vi "VIH Dialog - Project File List.vi"(4 "Ena Custom VI (F)":bool, 6 "File set (All)":enum32{"ALL", "conpane", "invalid"}(ring), 7 "Called from Master (F)":bool, 10 "Disable not buildable":bool, 11 "Project Tree":T2) -> (0 "OK out":bool, 2 "File Paths":path[](array[path]), 3 "File Path":path)   [LabVIEW 2014]
doc: "::: VI Helpeks :::\nCopyright (c) 2000-2026 Konstantin Shifershteyn. All rights reserved."
uses:
  VIH Project Tree Typedef - Tree Refnum.ctl
  _VIH HelpGen - Palette.llb/VIH HelpGen Typedef - Palette - Item Type Enum.ctl
  VIH Project Tree Typedef - Tree Item Type.ctl
  <vilib>/Utility/miscctls.llb/LVRowAndColumnUnsignedTypeDef.ctl
panel:
  in  "QualifiedNames":bool caption="Show qualified VI names"
  in  "KindOfFile":T1(ring) caption="Category Selector"
  in  "Files w NotFound Attrib":path[](array[path])
  in  "DirectSortColumn":i32
  in  "Files tmp":path[](array[path])
  in  "FileList":i32[](listbox) caption="File List"
  out "Sel Path":path caption="File Path"
  in  "%Arbitrary":bool caption="Custom VI"
  in  "%OK":bool caption="OK"
  in  "%Cancel":bool caption="Cancel"
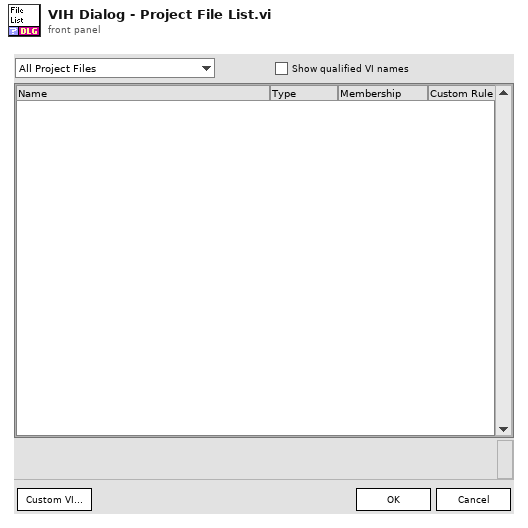
[diagram p1: front panel]
types:
  T1 = enum16{"All Project Files", "Palette menus", "Instruments (VI,VIT)", "VIs with Connector Pane", "Express VIs", "Polymorphic VIs", "Controls (CTL,CTT)", "HTML Files", "Other Files", "Invalid Files"}
  T2 = typedef "VIH Project Tree Typedef - Tree Refnum.ctl" = refnum<vi>
  T3 = typedef "VIH HelpGen Typedef - Palette - Item Type Enum.ctl" = enum32{"<Invalid>", "<unknown>", "VI", "Menu", "LV Func", "Express VI", "Poly VI", "CTL", "HTML"}
  T4 = cluster{"Types":T3[], "Paths":path[], "Dynamic":enum16{"Dyn", "Stat", "Both"}[], "Can be built":bool[], "Has rule":bool[], "Names":string[]}
  T5 = enum8{"Enabled", "Disabled", "Disabled and Grayed Out"}
  T6 = typedef "VIH Project Tree Typedef - Tree Item Type.ctl" = enum32{"<Invalid>", "Project", "Proj Files", "Proj Rules", "File Group", "Rule Group", "Any File", "LV Func", ".mnu", ".mnu (dyn)", ".vi", ".vi (dyn)", ".vit", ".vit (dyn)", ".ctl", ".ctl (dyn)", ".ctt", ".ctt (dyn)", "polyVI", "polyVI (dyn)", "expVI", "expVI (dyn)", "HTML", "PolyVI Inst"}
  T7 = typedef "LVRowAndColumnUnsignedTypeDef.ctl" = cluster{"Row":u32, "Column":u32}
  T8 = typedef "LVPoint32TypeDef.ctl" = cluster{"Horizontal":i32, "Vertical":i32}
  T9 = typedef "LVRowAndColumnTypeDef.ctl" = cluster{"Row":i32, "Column":i32}
  T10 = typedef "lveventtype.ctl" = enum32{"Null", "Timeout", "Annotation Menu Selection", "Annotation Menu Selection?", "App Instance Close", "App Instance Close?", "Autoscale Range Change", "Bookmark Info Change", "Cell Edit", "Cell Edit?", "Cursor Grab", "Cursor Grab?", "Cursor Menu Selection", "Cursor Menu Selection?", "Cursor Move", "Cursor Release", "Data Change", "Direction Change", "Display State Change", "Drag Ended", "Drag Enter", "Drag Leave", "Drag Over", "Drag Source Update", "Drag Starting", "Drag Starting?", "Drop", "Exec State Change", "Key Down", "Key Down?", "Key Repeat", "Key Repeat?", "Key Up", "Listbox Double Click", "Menu Activation?", "Menu Selection (App)", "Menu Selection? (App)", "Menu Selection (User)", "Mouse Down", "Mouse Down?", "Mouse Enter", "Mouse Leave", "Mouse Move", "Mouse Up", "Mouse Wheel", "NI Security User Change (App)", "Pane Size", "Panel Close", "Panel Close?", "Panel Resize", "Plot Attribute Change", "Scale Range Change", "Shortcut Menu Activation?", "Shortcut Menu Selection (App)", "Shortcut Menu Selection? (App)", "Shortcut Menu Selection (User)", "Tree Double Click", "Tree Drag", "Tree Drag?", "Tree Drop", "Tree Drop?", "Tree Item Close", "Tree Item Close?", "Tree Item Open", "Tree Item Open?", "User Event", "Value Change"}
  T11 = cluster{"Types":T3[], "Paths":path[], "Dynamic":enum16{"Dyn", "Stat", "Both"}[], "Can be built":bool[], "DynFileNotFound":bool[]}
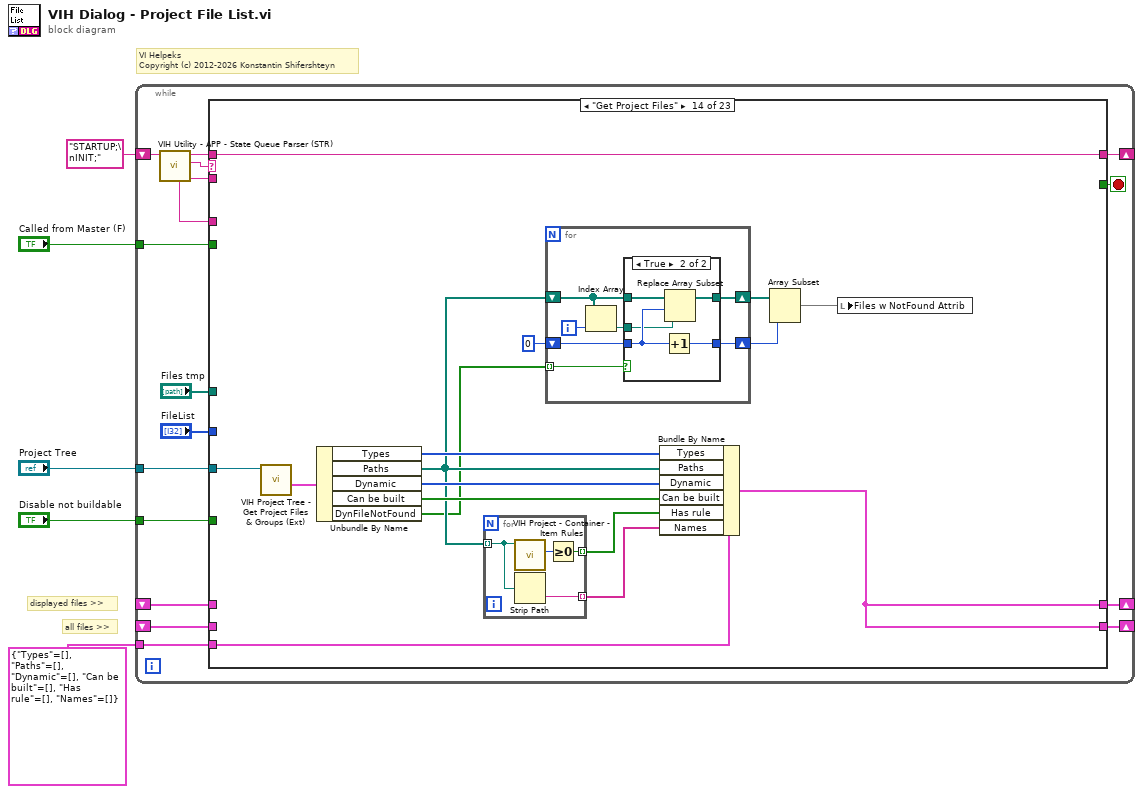
[diagram p0: block diagram]
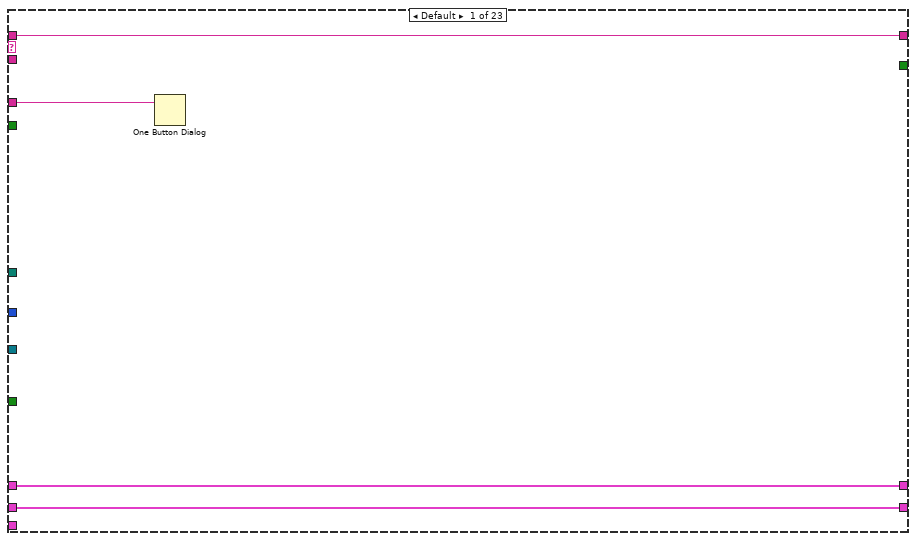
[diagram p2: hidden frame]
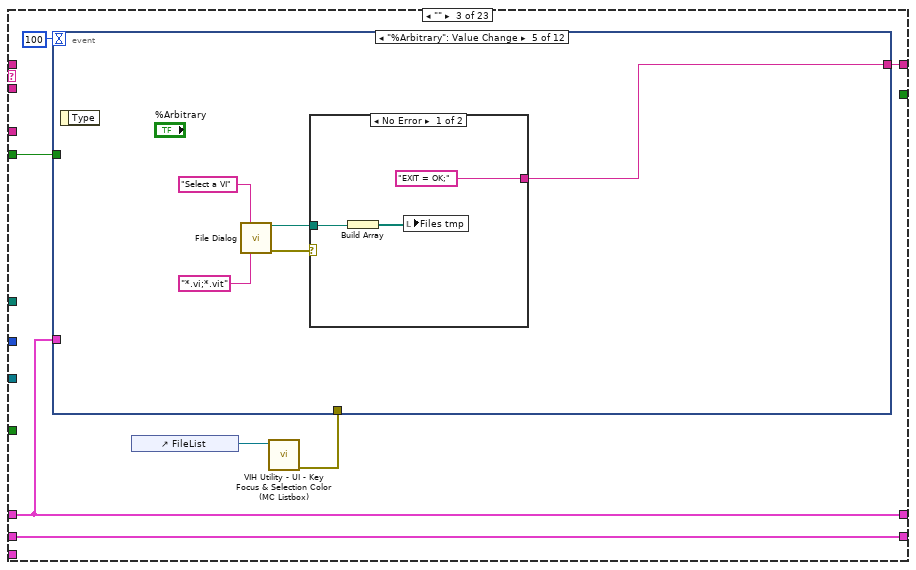
[diagram p4: hidden frame]
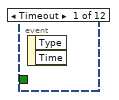
[diagram p5: hidden frame]
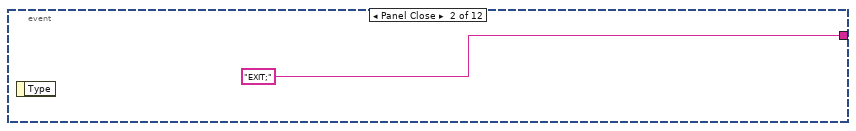
[diagram p6: hidden frame]
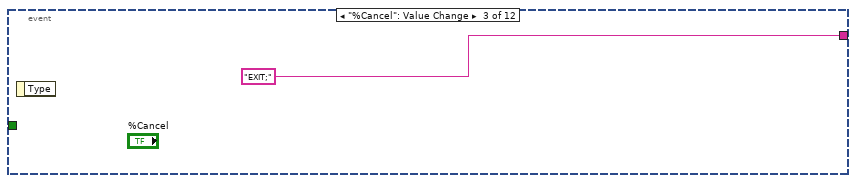
[diagram p7: hidden frame]
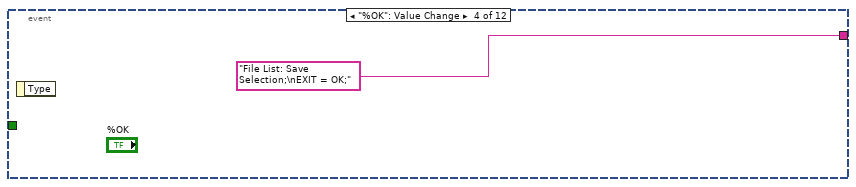
[diagram p8: hidden frame]
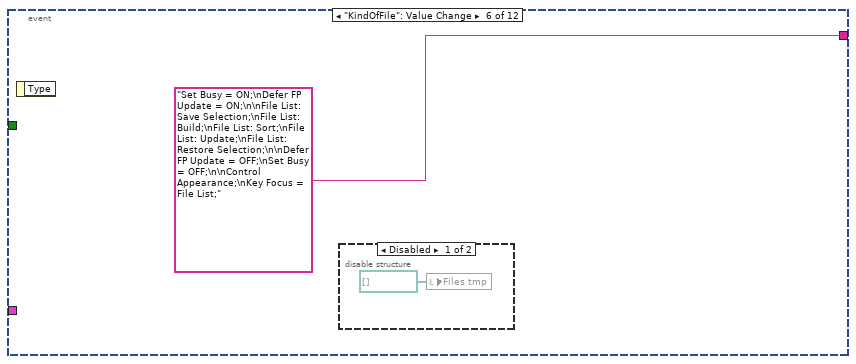
[diagram p10: hidden frame]
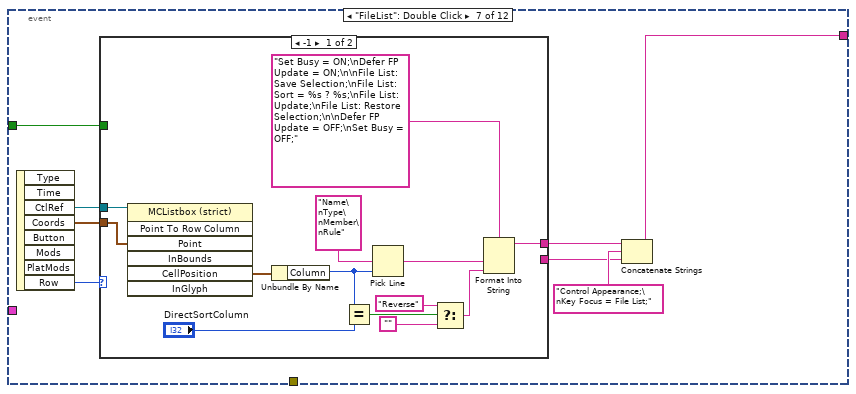
[diagram p12: hidden frame]
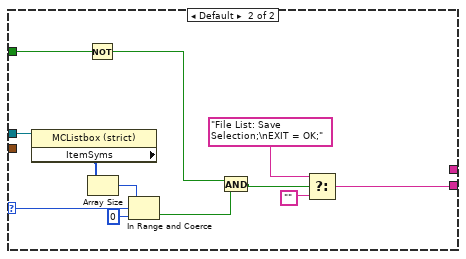
[diagram p13: hidden frame]
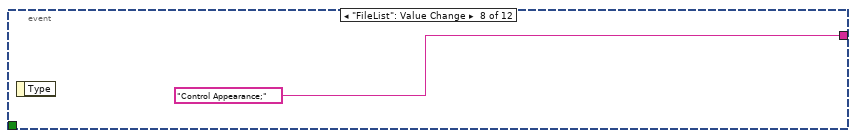
[diagram p14: hidden frame]
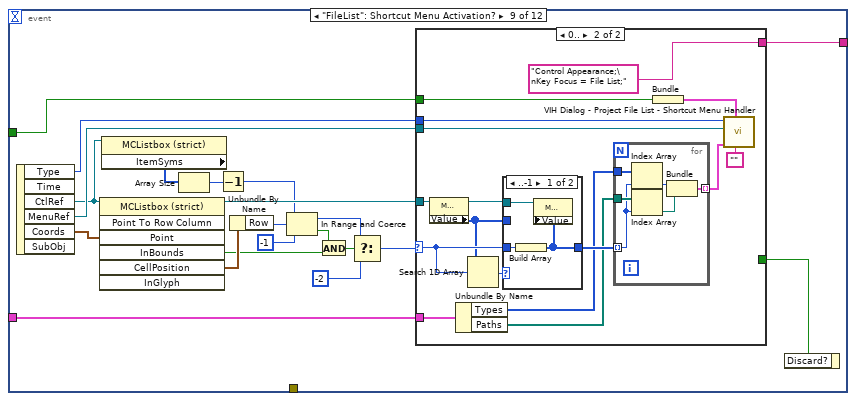
[diagram p15: hidden frame]
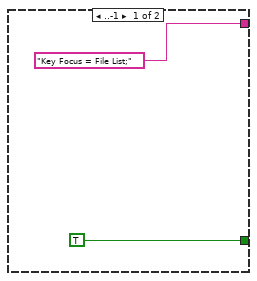
[diagram p16: hidden frame]
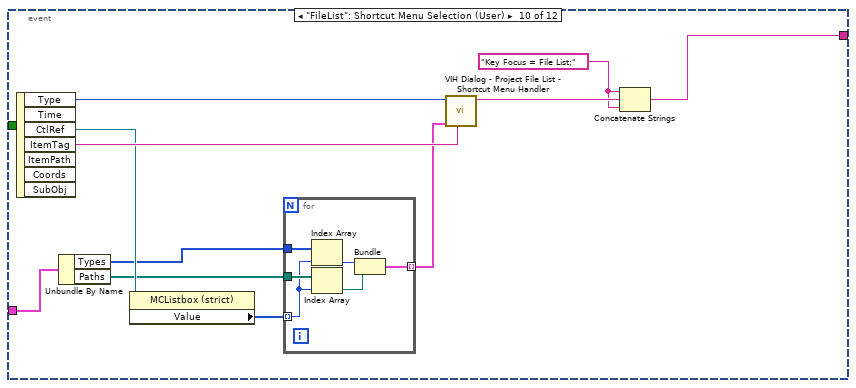
[diagram p18: hidden frame]
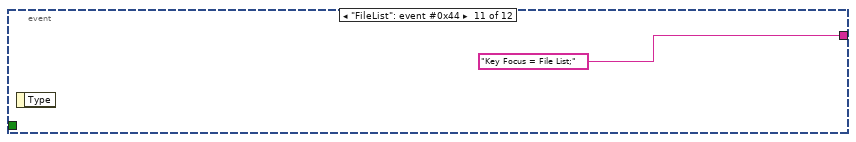
[diagram p19: hidden frame]
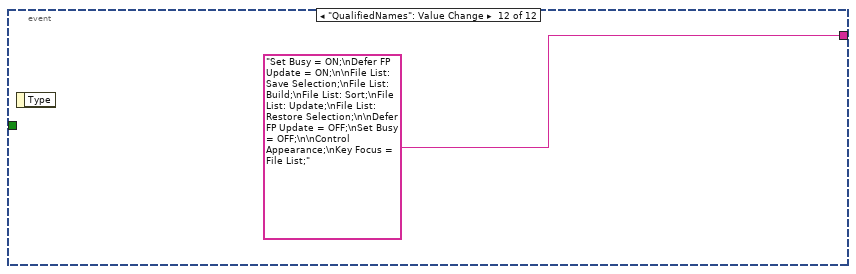
[diagram p20: hidden frame]
diagram:
  # "VI Helpeks\nCopyright (c) 2012-2026 Konstantin Shifershteyn"
  # "displayed files >>"
  # "all files >>"
  n1 = while {
    shift-right: [w20] -> _
    shift-left: "STARTUP;\nINIT;" -> [w22]
    tunnel: "Project Tree" -> [w15]
    shift-right: [w14] -> _
    shift-left: _ -> [w13]
    shift-right: [w12] -> _
    shift-left: _ -> [w11]
    tunnel: T4 {"Types"=[], "Paths"=[], "Dynamic"=[], "Can be built"=[], "Has rule"=[], "Names"=[]} ("Project Files") -> [w8]
    tunnel: "Called from Master (F)" -> [w7]
    tunnel: "Disable not buildable" -> [w6]
    stop <- w17 stop-if-true
    n2 = call "VIH Utility - APP - State Queue Parser (STR).vi"("input queue"=w22) -> ("state parameters"=w16:string, "state"=w21:string, "remained queue"=w19:string, "complete state specifier"=w18:string)  [unwired: 5 in]
    n3 = case shown="\"Get Project Files\"" w21 {
      tunnel: [w26 w29 w35 w153 w190 "File List: Clear;\nHALT;" w223 w237 w241 w247 w252 w264 w273 w289 w334 w453 w647 w717 w736 w756 w760 w767 w797] -> w20
      tunnel: w19 -> [w26 w29 _ w156 w191 _ w223 w237 w241 w247 w252 w264 w273 w289 w334 w453 w647 w717 w736 w756 w760 w775 w803]
      tunnel: w18 -> [w25 _ _ _ _ _ _ _ _ _ _ _ _ _ _ _ _ _ _ _ _ _ _]
      tunnel: [_ _ _ _ _ _ TRUE _ _ _ _ _ _ _ _ _ _ _ _ _ _ _ _] -> w17
      tunnel: w16 -> [_ _ _ _ _ w203 _ _ w238 w242 w249 _ _ _ _ w439 _ _ _ _ _ w771 w790]
      tunnel: w15 -> [_ _ _ _ _ _ _ _ _ _ _ _ _ w288 _ _ _ _ _ _ _ w772 w800]
      tunnel: [w24 w28 w34 w158 w188 w201 w221 w235 w239 w245 w250 w263 w271 w284 w333 w454 w648 w718 w737 w757 w758 w773 w801] -> w14
      tunnel: w13 -> [w24 w28 w34 w158 w188 w201 _ w235 w239 w245 w250 w263 w271 _ w333 w454 w648 w718 w737 w757 w758 w773 w801]
      tunnel: [w23 w27 w33 w157 w187 w198 w221 w236 w240 w246 w251 w262 w272 w284 w326 w447 w646 w716 w735 w755 w759 w774 w802] -> w12
      tunnel: w11 -> [w23 w27 w33 w157 w187 w198 _ w236 w240 w246 w251 w262 w272 _ _ w452 w646 w716 w735 w755 w759 w774 w802]
      tunnel: "FileList" -> [_ _ _ _ _ w197 _ _ _ _ _ w261 _ _ _ _ _ w715 _ _ _ _ _]
      tunnel: "Files tmp" -> [_ _ _ _ _ w200 _ _ _ _ _ _ _ _ _ _ _ _ w722 _ _ _ _]
      tunnel: w8 -> [_ _ _ _ _ _ w221 _ _ _ _ _ _ w286 w319 w444 _ _ _ _ _ _ _]
      tunnel: w7 -> [_ _ w32 _ w173 _ _ _ _ _ _ w257 _ _ _ _ _ _ _ _ _ _ _]
      tunnel: w6 -> [_ _ _ _ _ _ _ _ _ _ _ _ _ _ _ _ w632 _ _ _ _ _ _]
      frame Default {
        n4 = One Button Dialog(message=w25) -> ()  [unwired: 1 in, 1 out]
      }
      frame "#" {
      }
      frame "" {
        n5 = control-ref of="FileList"() -> (w31:refnum<vi>)
        n6 = call "VIH Utility - UI - Key Focus & Selection Color (MC Listbox).vi"("MCListbox Refnum"=w31) -> ("error out"=w30:errorcluster)  [unwired: 8 in, 2 out]
        n7 = event shown="[4] \"%Arbitrary\": Value Change" {
          selector: _ -> [_ _ _ _ _ _ _ _ _ _ _ _]
          dyn-events: _ -> [_ _ _ _ _ _ _ _ _ _ _ _]
          timeout: 100 -> [_ _ _ _ _ _ _ _ _ _ _ _]
          tunnel: [_ "EXIT;" "EXIT;" "File List: Save Selection;\nEXIT = OK;" w40 "Set Busy = ON;\nDefer FP Update = ON;\n\nFile List: Save Selection;\nFile List: Build;\nFile List: Sort;\nFile List: Update;\nFile List: Restore Selection;\n\nDefer FP Update = OFF;\nSet Busy = OFF;\n\nControl Appearance;\nKey Focus = File List;" w53 "Control Appearance;" w87 w136 "Key Focus = File List;" ("string") "Set Busy = ON;\nDefer FP Update = ON;\n\nFile List: Save Selection;\nFile List: Build;\nFile List: Sort;\nFile List: Update;\nFile List: Restore Selection;\n\nDefer FP Update = OFF;\nSet Busy = OFF;\n\nControl Appearance;\nKey Focus = File List;"] -> w35
          tunnel: w33 -> [_ _ _ _ _ _ _ _ w96 w138 _ _]
          tunnel: w32 -> [_ _ _ _ _ _ w50 _ w95 _ _ _]
          tunnel: w30 -> [_ _ _ _ _ _ _ _ _ _ _ _]
          event Timeout {
            n8 = event-data() -> ()  [unwired: 1 in, 2 out]
          }
          event Panel Close {
            n9 = event-data() -> ()  [unwired: 1 in, 1 out]
          }
          event "%Cancel": Value Change {
            n10 = event-data() -> ()  [unwired: 1 in, 1 out]
          }
          event "%OK": Value Change {
            n11 = event-data() -> ()  [unwired: 1 in, 1 out]
          }
          event "%Arbitrary": Value Change {
            n12 = event-data() -> ()  [unwired: 1 in, 1 out]
            n13 = call "File Dialog"("prompt"="Select a VI", "pattern (all files)"="*.vi;*.vit") -> ("selected path"=w41:path, "error out"=w42:errorcluster)  [unwired: 10 in, 2 out]
            n14 = case shown="No Error" w42 {
              tunnel: w41 -> [w47 _]
              tunnel: ["EXIT = OK;" _] -> w40
              frame No Error {
                n15 = Build Array(w47) -> (w46:path[])
                n16 = local write "Files tmp"(w46) -> ()
              }
              frame Error {
              }
            }
          }
          event "KindOfFile": Value Change {
            n17 = event-data() -> ()  [unwired: 1 in, 1 out]
            n18 = disable-structure shown="Disabled" {
              frame Disabled {
                n19 = local write "Files tmp"(path[] [] ("Files tmp")) -> ()
              }
              frame Enabled {
              }
            }
          }
          event "FileList": Double Click {
            n20 = event-data() -> ("CtlRef"=w56:refnum<vi>, "Coords"=w55:T8, "Row"=w57:i32)  [unwired: 1 in, 5 out]
            n21 = case shown="-1" w57 {
              selector: w57 -> [_ w81]
              tunnel: w56 -> [w70 w82]
              tunnel: w55 -> [w69 _]
              tunnel: [w64 _] -> w54
              tunnel: [_ w77] -> w51
              tunnel: w50 -> [_ w72]
              frame -1 {
                n22 = invoke class="MCListbox (strict)" method="Point To Row Column"(reference=w70, "Point"=w69) -> ("CellPosition"=w68:T9)  [unwired: 5 in, 6 out]
                n23 = Unbundle By Name(w68) -> ("Column"=w62:i32)
                n24 = Equal?(x=w62, y="DirectSortColumn") -> (x = y?=w61:bool)
                n25 = Pick Line(multi-line string="Name\nType\nMember\nRule", line index=w62) -> (output string=w65:string)  [unwired: 1 in]
                n26 = Select(t="Reverse", s=w61, f="") -> (s? t:f=w59:string)
                n27 = Format Into String(format string="Set Busy = ON;\nDefer FP Update = ON;\n\nFile List: Save Selection;\nFile List: Sort = %s ? %s;\nFile List: Update;\nFile List: Restore Selection;\n\nDefer FP Update = OFF;\nSet Busy = OFF;", w65, w59) -> (resulting string=w64:string)  [unwired: 2 in, 1 out]
              }
              frame Default {
                n28 = property class="MCListbox (strict)"(reference=w82) -> ("ItemSyms"=w80:i32[])  [unwired: 1 in, 2 out]
                n29 = Not(x=w72) -> (.not. x?=w71:bool)
                n30 = Array Size(array=w80) -> (size(s)=w79:i32)
                n31 = In Range and Coerce(upper limit=w79, x=w81, lower limit=0) -> (In Range?=w73:bool)  [unwired: 1 out]
                n32 = And(x=w71, y=w73) -> (x .and. y?=w74:bool)
                n33 = Select(t="File List: Save Selection;\nEXIT = OK;", s=w74, f="") -> (s? t:f=w77:string)
              }
            }
            n34 = Concatenate Strings(w54, "Control Appearance;\nKey Focus = File List;", w51) -> (w53:string)
          }
          event "FileList": Value Change {
            n35 = event-data() -> ()  [unwired: 1 in, 1 out]
          }
          event "FileList": Shortcut Menu Activation? {
            n36 = event-data() -> ("Type"=w98:T10, "CtlRef"=w94:refnum<vi>, "MenuRef"=w97:refnum<k9>, "Coords"=w104:T8)  [unwired: 1 in, 2 out]
            n37 = invoke class="MCListbox (strict)" method="Point To Row Column"(reference=w94, "Point"=w104) -> (reference out=w99:refnum<vi>, "InBounds"=w85:bool, "CellPosition"=w103:T9)  [unwired: 5 in, 4 out]
            n38 = property class="MCListbox (strict)"(reference=w94) -> ("ItemSyms"=w92:i32[])  [unwired: 1 in, 2 out]
            n39 = Array Size(array=w92) -> (size(s)=w91:i32)
            n40 = Decrement(x=w91) -> (x-1=w90:i32)
            n41 = Unbundle By Name(w103) -> ("Row"=w93:i32)
            n42 = In Range and Coerce(upper limit=w90, x=w93, lower limit=-1) -> (coerced(x)=w88:i32, In Range?=w86:bool)
            n43 = And(x=w86, y=w85) -> (x .and. y?=w84:bool)
            n44 = Select(t=w88, s=w84, f=-2) -> (s? t:f=w101:i32)
            n45 = case shown="0.." w101 {
              selector: w101 -> [_ w119]
              tunnel: [TRUE _] -> w100
              tunnel: w99 -> [_ w122]
              tunnel: w98 -> [_ w118]
              tunnel: w97 -> [_ w117]
              tunnel: w96 -> [_ w112]
              tunnel: w95 -> [_ w111]
              tunnel: ["Key Focus = File List;" "Control Appearance;\nKey Focus = File List;"] -> w87
              frame ..-1 {
              }
              frame 0.. {
                n46 = property class="MCListbox (strict)"(reference=w122) -> (reference out=w121:refnum<vi>, "Value"=w115:i32[])  [unwired: 1 in, 1 out]
                n47 = Unbundle By Name(w112) -> ("Types"=w109:T3[], "Paths"=w113:path[])
                n48 = Search 1D Array(1D array=w115, element=w119) -> (index of element=w120:i32)  [unwired: 1 in]
                n49 = case shown="..-1" w120 {
                  tunnel: w121 -> [w131 _]
                  tunnel: w119 -> [w130 _]
                  tunnel: [w129 w132] -> w114
                  tunnel: w115 -> [_ w132]
                  frame ..-1 {
                    n50 = Build Array(w130) -> (w129:i32[])
                    n51 = property class="MCListbox (strict)"(reference=w131, "Value"=w129) -> ()  [unwired: 1 in, 2 out]
                  }
                  frame 0.. {
                  }
                }
                n52 = for {
                  tunnel: w114 -> [w126] mode=indexing
                  tunnel: w113 -> [w128]
                  tunnel: w109 -> [w127]
                  tunnel: [w123] -> w108 mode=indexing
                  n53 = Index Array(array=w127, index=w126) -> (element=w125:T3)
                  n54 = Index Array(array=w128, index=w126) -> (element=w124:path)
                  n55 = Bundle("Item/File Type"=w125, w124) -> (w123:cluster{"Item/File Type":T3, path})  [unwired: 1 in]
                }
                n56 = Bundle("Called from Master (F)"=w111) -> (w110:cluster{"Called from Master (F)":bool})  [unwired: 1 in]
                n57 = call "VIH Dialog - Project File List - Shortcut Menu Handler.vi"("Menu Tag"="", "Options"=w110, "Files"=w108, "MenuRef"=w117, "Event Type"=w118) -> ()  [unwired: 6 in, 1 out]
              }
            }
            n58 = event-data("Discard?"=w100) -> ()  [unwired: 1 in, 1 out]
          }
          event "FileList": Shortcut Menu Selection (User) {
            w133 = "Key Focus = File List;" ("string")
            n59 = event-data() -> ("Type"=w143:T10, "CtlRef"=w140:refnum<vi>, "ItemTag"=w141:string)  [unwired: 1 in, 4 out]
            n60 = Unbundle By Name(w138) -> ("Types"=w135:T3[], "Paths"=w137:path[])
            n61 = property class="MCListbox (strict)"(reference=w140) -> ("Value"=w139:i32[])  [unwired: 1 in, 2 out]
            n62 = for {
              tunnel: w139 -> [w144] mode=indexing
              tunnel: w137 -> [w149]
              tunnel: w135 -> [w148]
              tunnel: [w145] -> w134 mode=indexing
              n63 = Index Array(array=w148, index=w144) -> (element=w147:T3)
              n64 = Index Array(array=w149, index=w144) -> (element=w146:path)
              n65 = Bundle("Item/File Type"=w147, w146) -> (w145:cluster{"Item/File Type":T3, path})  [unwired: 1 in]
            }
            n66 = call "VIH Dialog - Project File List - Shortcut Menu Handler.vi"("Menu Tag"=w141, "Files"=w134, "Event Type"=w143) -> ("States spec"=w142:string)  [unwired: 8 in]
            n67 = Concatenate Strings(w133, w142, w133) -> (w136:string)
          }
          event "FileList": event #0x44 {
            n68 = event-data() -> ()  [unwired: 1 in, 1 out]
          }
          event "QualifiedNames": Value Change {
            n69 = event-data() -> ()  [unwired: 1 in, 1 out]
          }
        }
      }
      frame "STARTUP" {
        n70 = control-ref of="FileList"() -> (w155:refnum<vi>)
        n71 = disable-structure shown="Disabled" {
          disable-tunnel: w155 -> [w161 _]
          disable-tunnel: "Utility - Set Project Tree & List Icons.vi" ("Utility VI Name") -> [w160 _]
          frame Disabled {
            n72 = call "VIH Utility - DEV - Get DevTime Utility VIs Folder.vi"("Utility VI Name"=w160) -> ("error out"=w167:errorcluster, "Utility VIs Path"=w166:path)  [unwired: 8 in, 1 out]
            n73 = Open VI Reference(type specifier VI Refnum (for type only)=refnum<vi> refnum, vi path=w166, error in (no error)=w167) -> (vi reference=w169:refnum<vi>, error out=w170:errorcluster)  [unwired: 3 in]
            n74 = call-by-ref "?"(reference=w169, error in=w170, "MCListbox Refnum"=w161) -> (reference out=w164:refnum<vi>, error out=w165:errorcluster, "error out (MCList)"=w162:errorcluster)  [unwired: 9 in, 1 out]
            n75 = Close Reference(reference=w164, error in (no error)=w165) -> (error out=w159:errorcluster)
            n76 = Select(t=w159, s=w159, f=w162) -> (s? t:f=w163:errorcluster)
            n77 = call <vilib>:"Simple Error Handler.vi"("error in (no error)"=w163) -> ()  [unwired: 4 in, 5 out]
          }
          frame Enabled {
          }
        }
        n78 = Concatenate Strings("File List: Clear;" ("string"), w156) -> (w153:string)
      }
      frame "INIT" {
        w171 = path[] [] ("Files tmp")
        n79 = call "VIH Utility - UI - Boolean to Control Disable Status.vi"("Status in"="Ena Custom VI (F)") -> ("Control Disable if False"=w185:u8)  [unwired: 3 in, 1 out]
        n80 = Not(x=w173) -> (.not. x?=w174:bool)
        n81 = property on="%Arbitrary" class="Bool"("DisabledEnum"=w185, "Visible"="Ena Custom VI (F)") -> ()  [unwired: 2 in, 2 out]
        n82 = property on="%OK" class="Bool"("Visible"=w174) -> ()  [unwired: 2 in, 2 out]
        n83 = Select(t="Close", s=w173, f="Cancel") -> (s? t:f=w180:string)
        n84 = case shown="\"invalid\"" "File set (All)" {
          tunnel: [T1."All Project Files" ("KindOfFile") T1."VIs with Connector Pane" ("KindOfFile") T1."Invalid Files" ("KindOfFile")] -> w184
          tunnel: [_ T5."Disabled and Grayed Out" ("Disabled") _] -> w183
          frame "ALL" {
          }
          frame "conpane" {
          }
          frame "invalid" {
          }
        }
        n85 = Initialize Array(w180, 4 ("dimension size")) -> (w179:string[])
        n86 = Select(t="Project Files", s=w173, f="Select a Project File") -> (s? t:f=w175:string)
        n87 = local write "Files w NotFound Attrib"(w171) -> ()
        n88 = local write "Files tmp"(w171) -> ()
        n89 = property on="%Cancel" class="Bool"("Strings [4]"=w179) -> ()  [unwired: 2 in, 2 out]
        n90 = property class="VI"("Front Panel.Title"=w175) -> ()  [unwired: 2 in, 2 out]
        n91 = property on="KindOfFile" class="Enum (strict)"("DisabledEnum"=w183, "Value"=w184) -> ()  [unwired: 2 in, 2 out]
        n92 = Concatenate Strings("Set Busy = ON;\nDefer FP Update = ON;\n\nGet Project Files;\n\nFile List: Build;\nFile List: Sort;\nFile List: Update;\nFile List: Restore Selection;\n\nDefer FP Update = OFF;\nSet Busy = OFF;\n\nControl Appearance;\nKey Focus = File List;", w191) -> (w190:string)
      }
      frame "EXIT" {
        n93 = case shown="\"Find In Tree\"" w203 {
          tunnel: [_ TRUE TRUE] -> w202
          tunnel: w200 -> [_ w206 w213]
          tunnel: [_ w205 w212] -> w199
          tunnel: w198 -> [_ _ w211]
          tunnel: w197 -> [_ _ w209]
          tunnel: [_ _ w208] -> w196
          frame Default {
          }
          frame "OK" {
            n94 = Index Array(array=w206) -> (element=w205:path)  [unwired: 1 in]
          }
          frame "Find In Tree" {
            n95 = Unbundle By Name(w211) -> ("Paths"=w210:path[])
            n96 = Index Array(array=w213) -> (element=w212:path)  [unwired: 1 in]
            n97 = for {
              tunnel: w210 -> [w217]
              tunnel: w209 -> [w216] mode=indexing
              tunnel: [w215] -> w208 mode=indexing
              n98 = Index Array(array=w217, index=w216) -> (element=w215:path)
            }
          }
        }
        "OK out" <- w202
        "File Path" <- w199
        "File Paths" <- w196
      }
      frame "HALT" {
        n99 = Call Chain() -> (call chain=w220:string[])
        n100 = Array Size(array=w220) -> (size(s)=w219:i32)
        n101 = case shown="2.." w219 {
          tunnel: [_ TRUE] -> w218
          frame ..1 {
          }
          frame 2.. {
            n102 = for {
              N: 100 -> [_]
              stop <- w233 continue-if-true
              n103 = property class="VI"("Front Panel.Open"=FALSE ("Front Panel Window:Open")) -> ("Front Panel.Open"=w233:bool)  [unwired: 2 in, 2 out]
              n104 = Wait (ms)(milliseconds to wait=u32 10) -> ()  [unwired: 1 out]
            }
          }
        }
        n105 = stacked-sequence {
          tunnel: w218 -> [_]
          frame #0 {
            w224 = T5."Enabled" ("Disabled")
            w226 = TRUE ("Visible")
            n106 = Initialize Array("Cancel", 4 ("dimension size")) -> (w228:string[])
            n107 = property on="%OK" class="Bool"("DisabledEnum"=w224, "Visible"=w226) -> ()  [unwired: 2 in, 2 out]
            n108 = property on="%Cancel" class="Bool"("Strings [4]"=w228) -> ()  [unwired: 2 in, 2 out]
            n109 = property on="%Arbitrary" class="Bool"("DisabledEnum"=w224, "Visible"=w226) -> ()  [unwired: 2 in, 2 out]
            n110 = property on="KindOfFile" class="Enum (strict)"("DisabledEnum"=T5."Enabled" ("Disabled")) -> ()  [unwired: 2 in, 2 out]
          }
        }
      }
      frame "--------------------------- 1" {
      }
      frame "Set Busy" {
        n111 = case shown="\"ON\"" w238 {
          frame "OFF", Default {
            n112 = call <vilib>:"Unset Busy.vi"() -> ()  [unwired: 11 in, 1 out]
          }
          frame "ON" {
            n113 = call <vilib>:"Set Busy.vi"() -> ()  [unwired: 10 in, 2 out]
          }
        }
      }
      frame "Defer FP Update" {
        n114 = case shown="\"ON\"" w242 {
          tunnel: [_ TRUE] -> w244
          frame "OFF", Default {
          }
          frame "ON" {
          }
        }
        n115 = property class="VI"() -> ("Front Panel"=w243:refnum<vi>)  [unwired: 2 in, 2 out]
        n116 = property class="Pnl"(reference=w243, "Defer Panel Updates"=w244) -> ()  [unwired: 1 in, 2 out]
      }
      frame "Key Focus" {
        n117 = case shown="\"File List\"" w249 {
          frame Default {
          }
          frame "File List" {
            n118 = control-ref of="FileList"() -> (w254:refnum<vi>)
            n119 = call "VIH Utility - UI - Key Focus & Selection Color (MC Listbox).vi"("F:Test/T:Set Key Focus (F)"=TRUE, "MCListbox Refnum"=w254) -> ()  [unwired: 7 in, 3 out]
          }
        }
      }
      frame "Control Appearance" {
        n120 = Array Size(array=w261) -> (size(s)=w259:i32)
        n121 = case shown="1" w259 {
          tunnel: w262 -> [_ w270]
          tunnel: w261 -> [_ w268]
          tunnel: [_ w266] -> w260
          tunnel: [TRUE _] -> w256
          frame Default {
          }
          frame 1 {
            n122 = Unbundle By Name(w270) -> ("Paths"=w269:path[])
            n123 = Index Array(array=w268) -> (element=w267:i32)  [unwired: 1 in]
            n124 = Index Array(array=w269, index=w267) -> (element=w266:path)
          }
        }
        "Sel Path" <- w260
        n125 = Or(x=w257, y=w256) -> (x .or. y?=w255:bool)
        n126 = call "VIH Utility - UI - Boolean to Control Disable Status.vi"("Status in"=w255) -> ("Control Disable if True"=w258:u8)  [unwired: 3 in, 1 out]
        n127 = property on="%OK" class="Bool"("DisabledEnum"=w258) -> ()  [unwired: 2 in, 2 out]
      }
      frame "--------------------------- 2" {
      }
      frame "Get Project Files" {
        n128 = call "VIH Project Tree - Get Project Files & Groups (Ext).vi"("Project Tree"=w288) -> ("Project Files"=w287:T11)  [unwired: 7 in, 3 out]
        n129 = Unbundle By Name(w287) -> ("Types"=w280:T3[], "Paths"=w279:path[], "Dynamic"=w285:enum16{"Dyn", "Stat", "Both"}[], "Can be built"=w282:bool[], "DynFileNotFound"=w277:bool[])
        n130 = for {
          tunnel: w279 -> [w305] mode=indexing
          tunnel: [w306] -> w283 mode=indexing
          tunnel: [w304] -> w281 mode=indexing
          n131 = call "VIH Project - Container - Item Rules.vi"("Item Path"=w305) -> ("Item Idx out"=w307:i32)  [unwired: 6 in, 4 out]
          n132 = Strip Path(path=w305) -> (name=w304:string)  [unwired: 1 out]
          n133 = Greater Or Equal To 0?(x=w307) -> (x >= 0?=w306:bool)
        }
        n134 = for {
          shift-right: [w296] -> w276
          shift-left: w279 -> [w292]
          shift-right: [w294] -> w275
          shift-left: 0 -> [w295]
          tunnel: w277 -> [w290] mode=indexing
          i -> [w293]
          n135 = Index Array(array=w292, index=w293) -> (element=w291:path)
          n136 = case shown="True" w290 {
            tunnel: w292 -> [w298 w303]
            tunnel: [w298 w302] -> w296
            tunnel: w295 -> [w297 w301]
            tunnel: [w297 w300] -> w294
            tunnel: w291 -> [_ w299]
            frame False {
            }
            frame True {
              n137 = Increment(x=w301) -> (x+1=w300:i32)
              n138 = Replace Array Subset(array=w303, new element=w299, index=w301) -> (w302:path[])
            }
          }
        }
        n139 = Bundle By Name(cluster=w286, "Types"=w280, "Paths"=w279, "Dynamic"=w285, "Can be built"=w282, "Has rule"=w283, "Names"=w281) -> (w284:T4)
        n140 = Array Subset(array=w276, length=w275) -> (w274:path[])  [unwired: 1 in]
        n141 = local write "Files w NotFound Attrib"(w274) -> ()
      }
      frame "File List: Build" {
        (unwired) VIH_HelpGen_Typedef_-_Palette_-_Item_Type_Enum."VI" ("element")
        n142 = Unbundle(w333) -> ("Types"=w323:T3[], "Paths"=w332:path[], "Dynamic"=w322:enum16{"Dyn", "Stat", "Both"}[], "Can be built"=w318:bool[], "Has rule"=w315:bool[], "Names"=w312:string[])
        n143 = Array Size(array=w323) -> (size(s)=w324:i32)
        n144 = for {
          N: w324 -> [_]
          shift-right: [w353] -> w330
          shift-left: w323 -> [w354]
          shift-right: [w352] -> w329
          shift-left: w332 -> [w351]
          shift-right: [w350] -> w310
          shift-left: 0 -> [w349]
          tunnel: "KindOfFile" -> [w347]
          shift-right: [w345] -> w321
          shift-left: w322 -> [w346]
          shift-right: [w343] -> w317
          shift-left: w318 -> [w344]
          shift-right: [w342] -> w314
          shift-left: w315 -> [w341]
          shift-right: [w339] -> w311
          shift-left: w312 -> [w340]
          tunnel: "QualifiedNames" -> [w335]
          i -> [w348]
          n145 = Index Array(array=w354, index=w348) -> (element=w338:T3)
          n146 = case shown="\"Other Files\"" w347 {
            tunnel: [TRUE w394 w397 w402 w406 w409 w412 w415 w418 w421] -> w355
            tunnel: w338 -> [_ w395 w398 w403 w407 w410 w413 w416 w419 w422]
            frame "All Project Files" {
            }
            frame "Palette menus" {
              n147 = case shown="\"Menu\"" w395 {
                tunnel: [_ TRUE] -> w394
                frame Default {
                }
                frame "Menu" {
                }
              }
            }
            frame "Instruments (VI,VIT)" {
              n148 = case shown="\"VI\"" w398 {
                tunnel: [_ TRUE TRUE TRUE] -> w397
                frame Default {
                }
                frame "VI" {
                }
                frame "Express VI" {
                }
                frame "Poly VI" {
                }
              }
            }
            frame "VIs with Connector Pane" {
              n149 = case shown="\"VI\"" w403 {
                tunnel: [_ TRUE TRUE] -> w402
                frame Default {
                }
                frame "VI" {
                }
                frame "Express VI" {
                }
              }
            }
            frame "Express VIs" {
              n150 = case shown="\"Express VI\"" w407 {
                tunnel: [_ TRUE] -> w406
                frame Default {
                }
                frame "Express VI" {
                }
              }
            }
            frame "Polymorphic VIs" {
              n151 = case shown="\"Poly VI\"" w410 {
                tunnel: [_ TRUE] -> w409
                frame Default {
                }
                frame "Poly VI" {
                }
              }
            }
            frame "Controls (CTL,CTT)" {
              n152 = case shown="\"CTL\"" w413 {
                tunnel: [_ TRUE] -> w412
                frame Default {
                }
                frame "CTL" {
                }
              }
            }
            frame "HTML Files" {
              n153 = case shown="\"HTML\"" w416 {
                tunnel: [_ TRUE] -> w415
                frame Default {
                }
                frame "HTML" {
                }
              }
            }
            frame "Other Files" {
              n154 = case shown="\"<unknown>\"" w419 {
                tunnel: [_ TRUE] -> w418
                frame Default {
                }
                frame "<unknown>" {
                }
              }
            }
            frame "Invalid Files" {
              n155 = case shown="\"<Invalid>\"" w422 {
                tunnel: [_ TRUE] -> w421
                frame Default {
                }
                frame "<Invalid>" {
                }
              }
            }
          }
          n156 = case shown="\"VI\"" w338 {
            tunnel: [_ _ TRUE _ _ TRUE TRUE TRUE _] -> w337
            frame "<Invalid>" {
            }
            frame "<unknown>" {
            }
            frame "VI" {
            }
            frame "Menu" {
            }
            frame "LV Func" {
            }
            frame "Express VI" {
            }
            frame "Poly VI" {
            }
            frame "CTL" {
            }
            frame "HTML" {
            }
          }
          n157 = And(x=w337, y=w335) -> (x .and. y?=w336:bool)
          n158 = case shown="True" w355 {
            tunnel: w354 -> [w366 w387]
            tunnel: [w366 w386] -> w353
            tunnel: [w365 w388] -> w352
            tunnel: w351 -> [w365 w383]
            tunnel: [w364 w385] -> w350
            tunnel: w349 -> [w364 w373]
            tunnel: w338 -> [_ w384]
            tunnel: w348 -> [_ w370]
            tunnel: w346 -> [w363 w381]
            tunnel: [w363 w380] -> w345
            tunnel: w344 -> [w362 w378]
            tunnel: [w362 w377] -> w343
            tunnel: [w361 w375] -> w342
            tunnel: w341 -> [w361 w374]
            tunnel: w340 -> [w360 w372]
            tunnel: [w360 w371] -> w339
            tunnel: w336 -> [_ w367]
            frame False {
            }
            frame True {
              n159 = Index Array(array=w383, index=w370) -> (element=w369:path)
              n160 = case shown="True" w367 {
                tunnel: w369 -> [w390 w392]
                tunnel: [w389 w391] -> w368
                frame False {
                  n161 = Strip Path(path=w390) -> (name=w389:string)  [unwired: 1 out]
                }
                frame True {
                  n162 = call "VIH HelpGen - FILE - Get Qualified Filename.vi"("File Path"=w392) -> ("Qualified name"=w391:string)  [unwired: 9 in, 1 out]
                }
              }
              n163 = Index Array(array=w381, index=w370) -> (element=w382:enum16{"Dyn", "Stat", "Both"})
              n164 = Index Array(array=w378, index=w370) -> (element=w379:bool)
              n165 = Index Array(array=w374, index=w370) -> (element=w376:bool)
              n166 = Replace Array Subset(array=w387, new element=w384, index=w373) -> (w386:T3[])
              n167 = Replace Array Subset(array=w383, new element=w369, index=w373) -> (w388:path[])
              n168 = Replace Array Subset(array=w381, new element=w382, index=w373) -> (w380:enum16{"Dyn", "Stat", "Both"}[])
              n169 = Replace Array Subset(array=w378, new element=w379, index=w373) -> (w377:bool[])
              n170 = Replace Array Subset(array=w374, new element=w376, index=w373) -> (w375:bool[])
              n171 = Replace Array Subset(array=w372, new element=w368, index=w373) -> (w371:string[])
              n172 = Increment(x=w373) -> (x+1=w385:i32)
            }
          }
        }
        n173 = Reshape Array(w330, w310) -> (w328:T3[])
        n174 = Reshape Array(w329, w310) -> (w327:path[])
        n175 = Reshape Array(w321, w310) -> (w320:enum16{"Dyn", "Stat", "Both"}[])
        n176 = Reshape Array(w317, w310) -> (w316:bool[])
        n177 = Reshape Array(w314, w310) -> (w313:bool[])
        n178 = Reshape Array(w311, w310) -> (w309:string[])
        n179 = Bundle(cluster=w319, "Types"=w328, "Paths"=w327, "Dynamic"=w320, "Can be built"=w316, "Has rule"=w313, "Names"=w309) -> (w326:T4)
      }
      frame "File List: Sort" {
        n180 = Unbundle(w452) -> ("Types"=w451:T3[], "Paths"=w450:path[], "Dynamic"=w446:enum16{"Dyn", "Stat", "Both"}[], "Can be built"=w443:bool[], "Has rule"=w441:bool[], "Names"=w426:string[])
        n181 = Match Pattern(string=w439, regular expression="\\?") -> (before substring=w437:string, after substring=w436:string)  [unwired: 1 in, 2 out]
        n182 = call <vilib>:"Trim Whitespace.vi"("string"=w437) -> ("trimmed string"=w435:string)  [unwired: 1 in]
        n183 = call <vilib>:"Trim Whitespace.vi"("string"=w436) -> ("trimmed string"=w429:string)  [unwired: 1 in]
        n184 = case shown="\"Name\", Default" w435 {
          tunnel: w451 -> [w487 w518 w563 w602]
          tunnel: w450 -> [w484 w519 w564 w603]
          tunnel: [w486 w521 w566 w605] -> w449
          tunnel: [w485 w520 w565 w604] -> w448
          tunnel: w446 -> [w483 w517 w561 w600]
          tunnel: [w482 w516 w562 w601] -> w445
          tunnel: w443 -> [w481 w515 w560 w598]
          tunnel: [w480 w514 w559 w599] -> w442
          tunnel: w441 -> [w479 w513 w558 w596]
          tunnel: [w478 w512 w557 w597] -> w440
          tunnel: [0 1 2 3] -> w427
          tunnel: w426 -> [w476 w509 w555 w593]
          tunnel: [w475 w510 w554 w594] -> w425
          frame "Name", Default {
            n185 = for {
              tunnel: w484 -> [w508] mode=indexing
              tunnel: [w505] -> w489 mode=indexing
              tunnel: w476 -> [w504] mode=indexing
              i -> [w507]
              n186 = To Lower Case(string=w504) -> (all lower case string=w506:string)
              n187 = Bundle(w506, w508, w507) -> (w505:cluster{string, path, i32})  [unwired: 1 in]
            }
            n188 = Sort 1D Array(array=w489) -> (sorted array=w488:cluster{string, path, i32}[])
            n189 = for {
              tunnel: w488 -> [w503] mode=indexing
              tunnel: w487 -> [w502]
              tunnel: w484 -> [w501]
              tunnel: [w500] -> w486 mode=indexing
              tunnel: [w499] -> w485 mode=indexing
              tunnel: w483 -> [w498]
              tunnel: [w497] -> w482 mode=indexing
              tunnel: w481 -> [w496]
              tunnel: [w495] -> w480 mode=indexing
              tunnel: w479 -> [w494]
              tunnel: [w493] -> w478 mode=indexing
              tunnel: w476 -> [w491]
              tunnel: [w490] -> w475 mode=indexing
              n190 = Unbundle(w503) -> (w492:i32)  [unwired: 2 out]
              n191 = Index Array(array=w502, index=w492) -> (element=w500:T3)
              n192 = Index Array(array=w501, index=w492) -> (element=w499:path)
              n193 = Index Array(array=w498, index=w492) -> (element=w497:enum16{"Dyn", "Stat", "Both"})
              n194 = Index Array(array=w496, index=w492) -> (element=w495:bool)
              n195 = Index Array(array=w494, index=w492) -> (element=w493:bool)
              n196 = Index Array(array=w491, index=w492) -> (element=w490:string)
            }
          }
          frame "Type" {
            n197 = for {
              tunnel: w519 -> [w544] mode=indexing
              tunnel: [w541] -> w523 mode=indexing
              tunnel: w518 -> [w540] mode=indexing
              tunnel: w509 -> [w538] mode=indexing
              i -> [w543]
              n198 = case shown="\"<Invalid>\"" w540 {
                tunnel: [-100 99 2 1 1000 10 9 20 50] -> w539
                frame "<Invalid>" {
                }
                frame "<unknown>" {
                }
                frame "VI" {
                }
                frame "Menu" {
                }
                frame "LV Func" {
                }
                frame "Express VI" {
                }
                frame "Poly VI" {
                }
                frame "CTL" {
                }
                frame "HTML" {
                }
              }
              n199 = To Lower Case(string=w538) -> (all lower case string=w542:string)
              n200 = Bundle(w539, w542, w544, w543) -> (w541:cluster{i32, string, path, i32})  [unwired: 1 in]
            }
            n201 = Sort 1D Array(array=w523) -> (sorted array=w522:cluster{i32, string, path, i32}[])
            n202 = for {
              tunnel: w522 -> [w537] mode=indexing
              tunnel: w518 -> [w536]
              tunnel: w519 -> [w535]
              tunnel: [w534] -> w521 mode=indexing
              tunnel: [w533] -> w520 mode=indexing
              tunnel: w517 -> [w532]
              tunnel: [w531] -> w516 mode=indexing
              tunnel: w515 -> [w530]
              tunnel: [w529] -> w514 mode=indexing
              tunnel: w513 -> [w528]
              tunnel: [w527] -> w512 mode=indexing
              tunnel: w509 -> [w526]
              tunnel: [w524] -> w510 mode=indexing
              n203 = Unbundle(w537) -> (w525:i32)  [unwired: 3 out]
              n204 = Index Array(array=w536, index=w525) -> (element=w534:T3)
              n205 = Index Array(array=w535, index=w525) -> (element=w533:path)
              n206 = Index Array(array=w532, index=w525) -> (element=w531:enum16{"Dyn", "Stat", "Both"})
              n207 = Index Array(array=w530, index=w525) -> (element=w529:bool)
              n208 = Index Array(array=w528, index=w525) -> (element=w527:bool)
              n209 = Index Array(array=w526, index=w525) -> (element=w524:string)
            }
          }
          frame "Member" {
            n210 = for {
              tunnel: w564 -> [w589] mode=indexing
              tunnel: [w586] -> w568 mode=indexing
              tunnel: w561 -> [w585] mode=indexing
              tunnel: w555 -> [w583] mode=indexing
              i -> [w588]
              n211 = case shown="\"Both\"" w585 {
                tunnel: [10 1 5] -> w584
                frame "Dyn" {
                }
                frame "Stat" {
                }
                frame "Both" {
                }
              }
              n212 = To Lower Case(string=w583) -> (all lower case string=w587:string)
              n213 = Bundle(w584, w587, w589, w588) -> (w586:cluster{i32, string, path, i32})  [unwired: 1 in]
            }
            n214 = Sort 1D Array(array=w568) -> (sorted array=w567:cluster{i32, string, path, i32}[])
            n215 = for {
              tunnel: w567 -> [w582] mode=indexing
              tunnel: w563 -> [w581]
              tunnel: w564 -> [w580]
              tunnel: [w579] -> w566 mode=indexing
              tunnel: [w578] -> w565 mode=indexing
              tunnel: w561 -> [w577]
              tunnel: [w576] -> w562 mode=indexing
              tunnel: w560 -> [w575]
              tunnel: [w574] -> w559 mode=indexing
              tunnel: w558 -> [w573]
              tunnel: [w572] -> w557 mode=indexing
              tunnel: w555 -> [w571]
              tunnel: [w570] -> w554 mode=indexing
              n216 = Unbundle(w582) -> (w569:i32)  [unwired: 3 out]
              n217 = Index Array(array=w571, index=w569) -> (element=w570:string)
              n218 = Index Array(array=w581, index=w569) -> (element=w579:T3)
              n219 = Index Array(array=w580, index=w569) -> (element=w578:path)
              n220 = Index Array(array=w577, index=w569) -> (element=w576:enum16{"Dyn", "Stat", "Both"})
              n221 = Index Array(array=w575, index=w569) -> (element=w574:bool)
              n222 = Index Array(array=w573, index=w569) -> (element=w572:bool)
            }
          }
          frame "Rule" {
            n223 = for {
              tunnel: w603 -> [w628] mode=indexing
              tunnel: [w625] -> w607 mode=indexing
              tunnel: w596 -> [w624] mode=indexing
              tunnel: w593 -> [w622] mode=indexing
              i -> [w627]
              n224 = Not(x=w624) -> (.not. x?=w623:bool)
              n225 = To Lower Case(string=w622) -> (all lower case string=w626:string)
              n226 = Bundle(w623, w626, w628, w627) -> (w625:cluster{bool, string, path, i32})  [unwired: 1 in]
            }
            n227 = Sort 1D Array(array=w607) -> (sorted array=w606:cluster{bool, string, path, i32}[])
            n228 = for {
              tunnel: w606 -> [w621] mode=indexing
              tunnel: w602 -> [w620]
              tunnel: w603 -> [w619]
              tunnel: [w618] -> w605 mode=indexing
              tunnel: [w617] -> w604 mode=indexing
              tunnel: w600 -> [w616]
              tunnel: [w615] -> w601 mode=indexing
              tunnel: w598 -> [w614]
              tunnel: [w613] -> w599 mode=indexing
              tunnel: w596 -> [w612]
              tunnel: [w611] -> w597 mode=indexing
              tunnel: w593 -> [w610]
              tunnel: [w609] -> w594 mode=indexing
              n229 = Unbundle(w621) -> (w608:i32)  [unwired: 3 out]
              n230 = Index Array(array=w620, index=w608) -> (element=w618:T3)
              n231 = Index Array(array=w619, index=w608) -> (element=w617:path)
              n232 = Index Array(array=w616, index=w608) -> (element=w615:enum16{"Dyn", "Stat", "Both"})
              n233 = Index Array(array=w614, index=w608) -> (element=w613:bool)
              n234 = Index Array(array=w612, index=w608) -> (element=w611:bool)
              n235 = Index Array(array=w610, index=w608) -> (element=w609:string)
            }
          }
        }
        n236 = case shown="Default" w429 {
          tunnel: w449 -> [w461 w474]
          tunnel: w448 -> [w460 w473]
          tunnel: w445 -> [w459 w472]
          tunnel: w442 -> [w458 w471]
          tunnel: w440 -> [w457 w470]
          tunnel: [w461 w469] -> w434
          tunnel: [w460 w468] -> w433
          tunnel: [w459 w467] -> w432
          tunnel: [w458 w466] -> w431
          tunnel: [w457 w465] -> w430
          tunnel: [w456 -1] -> w428
          tunnel: w427 -> [w456 _]
          tunnel: w425 -> [w455 w463]
          tunnel: [w455 w462] -> w424
          frame Default {
          }
          frame "Reverse" {
            n237 = Reverse 1D Array(array=w474) -> (reversed array=w469:T3[])
            n238 = Reverse 1D Array(array=w473) -> (reversed array=w468:path[])
            n239 = Reverse 1D Array(array=w472) -> (reversed array=w467:enum16{"Dyn", "Stat", "Both"}[])
            n240 = Reverse 1D Array(array=w471) -> (reversed array=w466:bool[])
            n241 = Reverse 1D Array(array=w470) -> (reversed array=w465:bool[])
            n242 = Reverse 1D Array(array=w463) -> (reversed array=w462:string[])
          }
        }
        n243 = local write "DirectSortColumn"(w428) -> ()
        n244 = Bundle(cluster=w444, "Types"=w434, "Paths"=w433, "Dynamic"=w432, "Can be built"=w431, "Has rule"=w430, "Names"=w424) -> (w447:T4)
      }
      frame "File List: Update" {
        n245 = Unbundle By Name(w646) -> ("Types"=w631:T3[], "Paths"=w630:path[], "Names"=w645:string[], "Dynamic"=w642:enum16{"Dyn", "Stat", "Both"}[], "Can be built"=w641:bool[], "Has rule"=w637:bool[])
        n246 = Array Size(array=w637) -> (size(s)=w638:i32)
        n247 = Initialize Array(0, w638) -> (w639:i32[])
        n248 = for {
          tunnel: w631 -> [w675] mode=indexing
          tunnel: [w674] -> w643 mode=indexing
          tunnel: w645 -> [w653] mode=indexing
          tunnel: [w672] -> w644 mode=indexing
          tunnel: w642 -> [w664] mode=indexing
          tunnel: w637 -> [w666] mode=indexing
          tunnel: w641 -> [w655] mode=indexing
          shift-right: [w660] -> w635
          shift-left: w639 -> [w661]
          shift-right: [w658] -> w634
          shift-left: 0 -> [w659]
          tunnel: w632 -> [w654]
          tunnel: w630 -> [w652] mode=indexing
          tunnel: "Files w NotFound Attrib" -> [w649]
          i -> [w657]
          n249 = case shown="\"<Invalid>\"" w675 {
            tunnel: [w687 w689 w692 VIH_Project_Tree_Typedef_-_Tree_Item_Type.".mnu (dyn)" ("Item Type") w700 VIH_Project_Tree_Typedef_-_Tree_Item_Type."expVI (dyn)" ("Item Type") VIH_Project_Tree_Typedef_-_Tree_Item_Type."polyVI (dyn)" ("Item Type") VIH_Project_Tree_Typedef_-_Tree_Item_Type.".ctl (dyn)" ("Item Type") w711] -> w671
            tunnel: ["<Invalid>" "File" "VI" "Palette" "Built In" "Express" "Polymorphic" "Control" "HTML"] -> w673
            tunnel: [w687 w689 VIH_Project_Tree_Typedef_-_Tree_Item_Type.".vi" ("Item Type") VIH_Project_Tree_Typedef_-_Tree_Item_Type.".mnu" ("Item Type") w700 VIH_Project_Tree_Typedef_-_Tree_Item_Type."expVI" ("Item Type") VIH_Project_Tree_Typedef_-_Tree_Item_Type."polyVI" ("Item Type") VIH_Project_Tree_Typedef_-_Tree_Item_Type.".ctl" ("Item Type") w711] -> w669
            tunnel: w655 -> [_ _ w694 _ _ _ _ _ _]
            frame "<Invalid>" {
              w687 = VIH_Project_Tree_Typedef_-_Tree_Item_Type."<Invalid>" ("Item Type")
            }
            frame "<unknown>" {
              w689 = VIH_Project_Tree_Typedef_-_Tree_Item_Type."Any File" ("Item Type")
            }
            frame "VI" {
              n250 = Select(t=VIH_Project_Tree_Typedef_-_Tree_Item_Type.".vi (dyn)" ("Item Type"), s=w694, f=VIH_Project_Tree_Typedef_-_Tree_Item_Type."PolyVI Inst") -> (s? t:f=w692:T6)
            }
            frame "Menu" {
            }
            frame "LV Func" {
              w700 = VIH_Project_Tree_Typedef_-_Tree_Item_Type."LV Func" ("Item Type")
            }
            frame "Express VI" {
            }
            frame "Poly VI" {
            }
            frame "CTL" {
            }
            frame "HTML" {
              w711 = VIH_Project_Tree_Typedef_-_Tree_Item_Type."HTML" ("Item Type")
            }
          }
          n251 = case shown="\"Dyn\"" w664 {
            tunnel: ["Dynamic" "Static" "Static & Dynamic"] -> w663
            tunnel: [TRUE _ _] -> w662
            frame "Dyn" {
            }
            frame "Stat" {
            }
            frame "Both" {
            }
          }
          n252 = Compound Arithmetic op=AND(invert w655, w654) -> (w656:bool)
          n253 = case shown="True" w656 {
            tunnel: w661 -> [w677 w682]
            tunnel: [w677 w681] -> w660
            tunnel: w659 -> [w676 w680]
            tunnel: [w676 w679] -> w658
            tunnel: w657 -> [_ w678]
            frame False {
            }
            frame True {
              n254 = Increment(x=w680) -> (x+1=w679:i32)
              n255 = Replace Array Subset(array=w682, new element=w678, index=w680) -> (w681:i32[])
            }
          }
          n256 = Search 1D Array(1D array=w649, element=w652) -> (index of element=w651:i32)  [unwired: 1 in]
          n257 = Select(t="Yes", s=w666, f="") -> (s? t:f=w665:string)
          n258 = Greater Or Equal To 0?(x=w651) -> (x >= 0?=w650:bool)
          n259 = Select(t=w671, s=w662, f=w669) -> (s? t:f=w670:T6)
          n260 = call "VIH Project Tree - Item Type to-from Icon Index.vi"("Not found"=w650, "Item Type"=w670) -> ("Icon Index out"=w674:i32)  [unwired: 9 in]
          n261 = Build Array(w653, w673, w663, w665) -> (w672:string[])
        }
        n262 = Reshape Array(w635, w634) -> (w633:i32[])
        n263 = property on="FileList" class="MCListbox (strict)"("ItemNames"=w644, "ItemSyms"=w643, "DisabledItems"=w633) -> ()  [unwired: 2 in, 2 out]
      }
      frame "File List: Save Selection" {
        n264 = Unbundle By Name(w716) -> ("Paths"=w714:path[])
        n265 = for {
          tunnel: w715 -> [w721] mode=indexing
          tunnel: w714 -> [w720]
          tunnel: [w719] -> w713 mode=indexing
          n266 = Index Array(array=w720, index=w721) -> (element=w719:path)
        }
        n267 = local write "Files tmp"(w713) -> ()
      }
      frame "File List: Restore Selection" {
        n268 = Unbundle By Name(w735) -> ("Paths"=w734:path[])
        n269 = Array Size(array=w722) -> (size(s)=w732:i32)
        n270 = Initialize Array(0, w732) -> (w731:i32[])
        n271 = for {
          tunnel: w734 -> [w744]
          tunnel: w722 -> [w743] mode=indexing
          shift-right: [w741] -> w729
          shift-left: w731 -> [w740]
          shift-right: [w739] -> w728
          shift-left: 0 -> [w738]
          n272 = Search 1D Array(1D array=w744, element=w743) -> (index of element=w742:i32)  [unwired: 1 in]
          n273 = case shown="0.." w742 {
            selector: w742 -> [_ w750]
            tunnel: [w746 w747] -> w741
            tunnel: w740 -> [w746 w751]
            tunnel: [w745 w748] -> w739
            tunnel: w738 -> [w745 w749]
            frame ..-1 {
            }
            frame 0.. {
              n274 = Replace Array Subset(array=w751, new element=w750, index=w749) -> (w747:i32[])
              n275 = Increment(x=w749) -> (x+1=w748:i32)
            }
          }
        }
        n276 = Reshape Array(w729, w728) -> (w727:i32[])
        n277 = Sort 1D Array(array=w727) -> (sorted array=w724:i32[])
        n278 = control-ref of="FileList"() -> (w726:refnum<vi>)
        n279 = property on="FileList" class="MCListbox (strict)"("Value"=w724) -> (error out=w725:errorcluster)  [unwired: 2 in, 1 out]
        n280 = Index Array(array=w724) -> (element=w723:i32)  [unwired: 1 in]
        n281 = call "VIH Utility - UI - Make Row Visible (MC Listbox).vi"("error in"=w725, "Row"=w723, "MC Listbox Refnum"=w726) -> ()  [unwired: 7 in, 2 out]
      }
      frame "File List: Clear" {
        w752 = i32[] [] ("Item Symbols")
        n282 = property on="FileList" class="MCListbox (strict)"("TopLeft"=T7 {"Row"=0, "Column"=0} ("Top Left Visible Cell"), "Value"=w752, "ItemNames"=string[][] [] ("Item Names"), "ItemSyms"=w752) -> ()  [unwired: 2 in, 2 out]
      }
      frame "--------------------------- 3" {
      }
      frame "Find File" {
        n283 = String To Path(string=w771) -> (path=w770:path)
        n284 = flat-sequence {
          tunnel: w770 -> [w776]
          tunnel: w772 -> [w777]
          tunnel: [w777] -> w764
          tunnel: [w776] -> w763
          tunnel: w764 -> [w781]
          tunnel: w763 -> [w780]
          tunnel: [w779] -> w762
          tunnel: [w778] -> w761
          tunnel: [w782] -> w765
          tunnel: [w783] -> w769
          tunnel: w762 -> [w783]
          tunnel: w761 -> [w782]
          frame #0 {
            n285 = call <vilib>:"Set Busy.vi"() -> ()  [unwired: 10 in, 2 out]
          }
          frame #1 {
            n286 = call "VIH Dialog - Find File on Disk.vi"("File Path"=w780, "Project Tree"=w781) -> ("New File Path"=w778:path, "New Tree Item Tag"=w779:string)  [unwired: 6 in, 2 out]
          }
          frame #2 {
            n287 = call <vilib>:"Unset Busy.vi"() -> ()  [unwired: 11 in, 1 out]
          }
        }
        n288 = Empty String/Path?(string/path=w769) -> (empty?=w768:bool)
        n289 = case shown="False" w768 {
          tunnel: ["Set Busy = ON;\nDefer FP Update = ON;\n\nGet Project Files;\n\nFile List: Build;\nFile List: Sort;\nFile List: Update;\nFile List: Restore Selection;\n\nDefer FP Update = OFF;\nSet Busy = OFF;\n\nControl Appearance;\nKey Focus = File List;" _] -> w766
          tunnel: w765 -> [w786 _]
          frame False {
            n290 = Build Array(w786) -> (w785:path[])
            n291 = local write "Files tmp"(w785) -> ()
          }
          frame True {
          }
        }
        n292 = Concatenate Strings(w766, w775) -> (w767:string)
      }
      frame "Search Files" {
        n293 = call "VIH Utility - STR - String to 1D Str Array.vi"("delimiter ('\\n')"="?" ("delimiter ('\\n')"), "String in"=w790) -> ("Array out"=w788:string[])  [unwired: 5 in]
        n294 = String To Path(string=w788) -> (path=w787:path[])
        n295 = flat-sequence {
          tunnel: w787 -> [w804]
          tunnel: w800 -> [w805]
          tunnel: [w805] -> w794
          tunnel: [w804] -> w793
          tunnel: w794 -> [w809]
          tunnel: w793 -> [w808]
          tunnel: [w807] -> w792
          tunnel: [w806] -> w791
          tunnel: [w810] -> w795
          tunnel: [w811] -> w799
          tunnel: w792 -> [w811]
          tunnel: w791 -> [w810]
          frame #0 {
            n296 = call <vilib>:"Set Busy.vi"() -> ()  [unwired: 10 in, 2 out]
          }
          frame #1 {
            n297 = call "VIH Dialog - Search Files in Folder.vi"("File Paths"=w808, "Project Tree"=w809) -> ("File Paths out"=w806:path[], "Tree Item Tags out"=w807:string[])  [unwired: 6 in, 2 out]
          }
          frame #2 {
            n298 = call <vilib>:"Unset Busy.vi"() -> ()  [unwired: 11 in, 1 out]
          }
        }
        n299 = Empty Array?(array=w799) -> (empty?=w798:bool)
        n300 = case shown="False" w798 {
          tunnel: ["Set Busy = ON;\nDefer FP Update = ON;\n\nGet Project Files;\n\nFile List: Build;\nFile List: Sort;\nFile List: Update;\nFile List: Restore Selection;\n\nDefer FP Update = OFF;\nSet Busy = OFF;\n\nControl Appearance;\nKey Focus = File List;" _] -> w796
          tunnel: w795 -> [w812 _]
          frame False {
            n301 = local write "Files tmp"(w812) -> ()
          }
          frame True {
          }
        }
        n302 = Concatenate Strings(w796, w803) -> (w797:string)
      }
    }
  }
